vi "CO move Mast.vi"(8 "error in (no error)":errorcluster caption="에러 입력(에러 없음)", 9 "Speed (1~8)":i32=1 min=1 max=8, 10 "Height (100~400)":i32=100 min=100 max=400, 11 "Instrument Manager 입력":refnum<class "Instrument Manager.lvclass">) -> (0 "error out":errorcluster caption="에러 출력", 3 "Instrument Manager 출력":refnum<class "Instrument Manager.lvclass">)   [LabVIEW 2023, in "Instrument Manager.lvclass"]
uses:
  Instrument Manager.lvclass
  Instrument Manager.lvclass/Instrument Manager.ctl
  Module/Turn Table and Mast Control/Class/CO3000/CO3000.lvclass
  Module/Turn Table and Mast Control/Interface Class/Mast/Interface - Mast.lvclass
  59d3c4a4-7653-4d1c-b38d-60c5a967f422.vi
  C:/Users/HCT-3320/Documents/Instrument Manger/Module/Turn Table and Mast Control/Class/CO3000/CO3000.lvclass
  C:/Users/HCT-3320/Documents/Instrument Manger/Module/Turn Table and Mast Control/Interface Class/Mast/Interface - Mast.lvclass
  C:/Users/HCT-3320/Documents/Instrument Manger/Module/Turn Table and Mast Control/Interface Class/Turn Table/Interface - Turn Table.lvclass
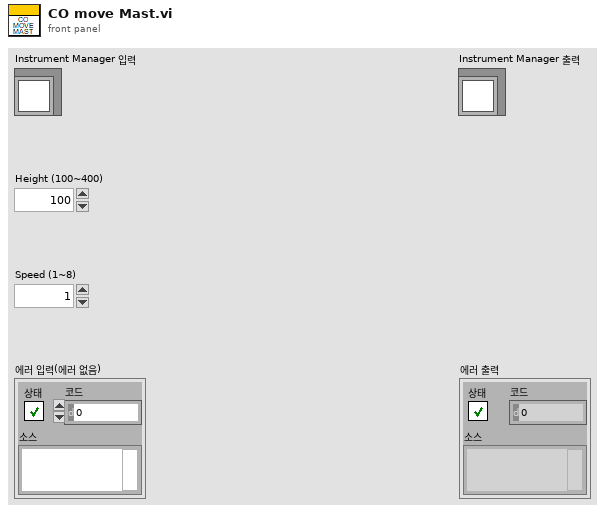
[diagram p1: front panel]
types:
  T1 = cluster{"Anritsu Call Box":refnum<class "Anritsu Call Box.lvclass">, "Spectrum Analyzer":refnum<class "Interface_Spectrum.lvclass">, "RF Switch Box":refnum<class "RF Filter Box.lvclass">, "Turn Table":refnum<class "Interface - Turn Table.lvclass">, "Mast":refnum<class "Interface - Mast.lvclass">, "3D Controller":refnum<class "Interface_3D Controller.lvclass">}
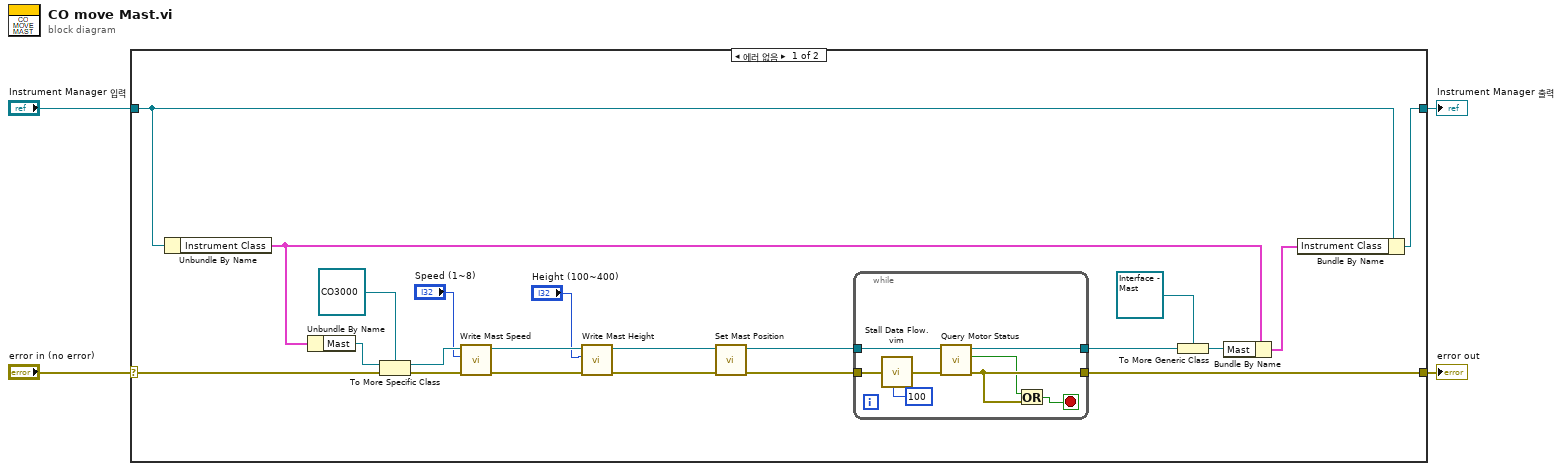
[diagram p0: block diagram]
diagram:
  n1 = case shown="에러 없음" "error in (no error)" {
    selector: "error in (no error)" -> [w23 w35]
    tunnel: [w5 w35] -> w3
    tunnel: [w11 w34] -> w1
    tunnel: "Instrument Manager 입력" -> [w12 w34]
    frame No Error {
      n2 = Unbundle By Name(w12) -> ("Instrument Class"=w21:T1)
      n3 = Unbundle By Name(w21) -> ("Mast"=w25:refnum<class "Interface - Mast.lvclass">)
      n4 = To More Specific Class(target class=refnum<class "CO3000.lvclass"> refnum ("Turn Table and Mast.lvlib:CO3000.lvclass"), reference=w25, error in=w23) -> (specific class reference=w19:refnum<class "CO3000.lvclass">, error out=w20:errorcluster)
      n5 = call "Write Mast Speed.vi"("error in (no error)"=w20, "Speed (1~8)"="Speed (1~8)", "CO3000 in"=w19) -> ("error out"=w18:errorcluster, "CO3000 out"=w16:refnum<class "CO3000.lvclass">)  [unwired: 7 in]
      n6 = call "Write Mast Height.vi"("error in (no error)"=w18, "Height (100~400)"="Height (100~400)", "CO3000 in"=w16) -> ("error out"=w17:errorcluster, "CO3000 out"=w15:refnum<class "CO3000.lvclass">)  [unwired: 7 in]
      n7 = call-dynamic "Set Mast Position.vi"("error in (no error)"=w17, "CO3000 in"=w15) -> ("error out"=w8:errorcluster, "CO3000 out"=w7:refnum<class "CO3000.lvclass">)  [unwired: 8 in]
      n8 = while {
        tunnel: w7 -> [w33]
        tunnel: w8 -> [w32]
        tunnel: [w28] -> w5
        tunnel: [w29] -> w6
        stop <- w26 stop-if-true
        n9 = call "Stall Data Flow.vim"("value in"=w32, "milliseconds to wait"=u32 100) -> ("value out"=w30:errorcluster)  [unwired: 1 out]
        n10 = call-dynamic "Query Motor Status.vi"("error in (no error)"=w30, "CO3000 in"=w33) -> ("error out"=w28:errorcluster, "Motor Stop?"=w27:bool, "CO3000 out"=w29:refnum<class "CO3000.lvclass">)  [unwired: 7 in]
        n11 = Or(x=w27, y=w28) -> (x .or. y?=w26:bool)
      }
      n12 = To More Generic Class(target class=refnum<class "Interface - Mast.lvclass"> refnum ("Turn Table and Mast.lvlib:Interface - Mast.lvclass"), reference=w6) -> (generic class reference=w14:refnum<class "Interface - Mast.lvclass">)
      n13 = Bundle By Name(cluster=w21, "Mast"=w14) -> (w13:T1)
      n14 = Bundle By Name(cluster=w12, "Instrument Class"=w13) -> (w11:refnum<class "Instrument Manager.lvclass">)
    }
    frame Error {
    }
  }
  "error out" <- w3
  "Instrument Manager 출력" <- w1
